vi "write.vi"(8 "error in (no error)":errorcluster, 10 "Angle(°)":dbl, 11 "rotationTable in":refnum<class "rotationTable.lvclass">) -> (0 "error out":errorcluster, 3 "rotationTable out":refnum<class "rotationTable.lvclass">)   [LabVIEW 2020, in "rotationTable.lvclass"]
uses:
  rotationTable.lvclass
  lexitekDriver_client/RPC Messages/frontend_message.ctl
  lexitekDriver_client/RPC Messages/backend_response.ctl
  rotationTable.lvclass/rotationTable.ctl
  lexitekDriver_client/lexitekDriver_client.lvlib
panel:
  out "Response Data":T1
  in  "Request Data":T2
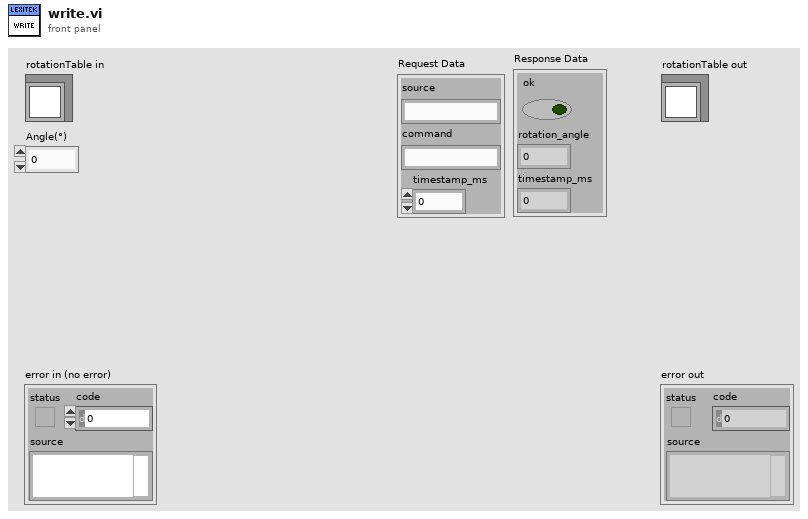
[diagram p1: front panel]
types:
  T1 = typedef "lexitekDriver_client.lvlib/backend_response.ctl" = cluster{"ok":bool, "rotation_angle":dbl, "timestamp_ms":u64}
  T2 = typedef "lexitekDriver_client.lvlib/frontend_message.ctl" = cluster{"source":string, "command":string, "timestamp_ms":u64}
  T3 = typedef "grpc-lvsupport-release.lvlib/grpcId.ctl" = u64
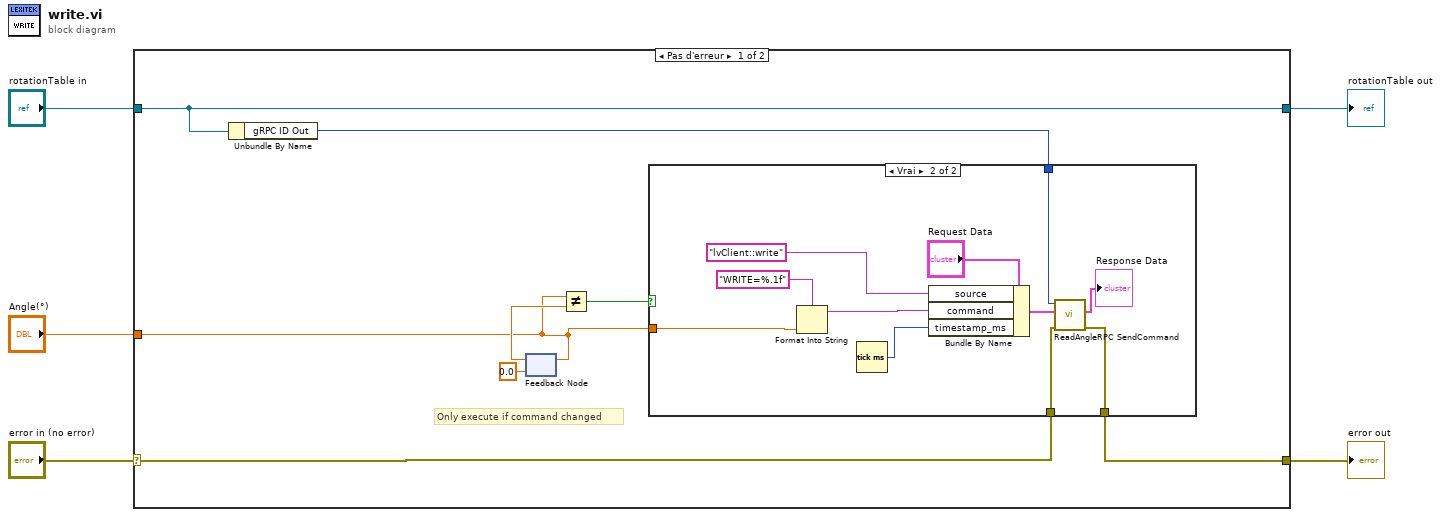
[diagram p0: block diagram]
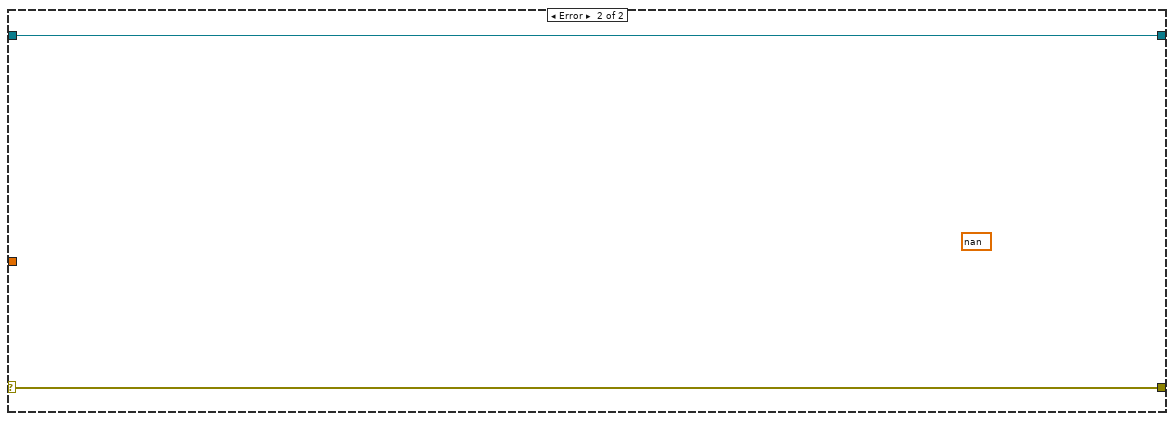
[diagram p3: hidden frame]
diagram:
  n1 = case shown="Pas d'erreur" "error in (no error)" {
    selector: "error in (no error)" -> [w7 w27]
    tunnel: [w12 w27] -> w4
    tunnel: [w13 w26] -> w2
    tunnel: "rotationTable in" -> [w13 w26]
    tunnel: "Angle(°)" -> [w9 _]
    frame No Error {
      # "Only execute if command changed"
      n2 = Unbundle By Name(w13) -> ("gRPC ID Out"=w6:T3)
      n3 = feedback-in #1(w9) -> ()
      n4 = feedback #1(0.0 ("Angle(°)")) -> (w10:dbl)
      n5 = Not Equal?(x=w9, y=w10) -> (x != y?=w8:bool)
      n6 = case shown="Vrai" w8 {
        tunnel: w6 -> [_ w20]
        tunnel: w7 -> [w14 w19]
        tunnel: [w14 w18] -> w12
        tunnel: w9 -> [_ w16]
        frame False {
        }
        frame True {
          n7 = Format Into String(format string="WRITE=%.1f" ("chaîne de format"), w16) -> (resulting string=w21:string)  [unwired: 2 in, 1 out]
          n8 = Tick Count (ms)() -> (millisecond timer value=w15:u32)
          n9 = Bundle By Name(cluster="Request Data", "source"="lvClient::write", "command"=w21, "timestamp_ms"=w15) -> (w24:T2)
          n10 = call "ReadAngleRPC SendCommand.vi"("error in"=w19, "Request Data"=w24, "gRPC ID"=w20) -> ("error out"=w18:errorcluster, "Response Data"=→"Response Data":T1)  [unwired: 6 in, 1 out]
        }
      }
    }
    frame Error {
      (unwired) nan ("rotation_angle")
    }
  }
  "error out" <- w4
  "rotationTable out" <- w2
